vi "DMM Measure Internal Resistance.vi"(0 "instrument handle":refnum<k15>, 5 "V1 (V)":dbl, 11 "error in":errorcluster) -> (4 "instrument handle out":refnum<k15>, 6 "Diode Voltage (V)":dbl, 8 "V2 (V)":dbl, 10 "Internal Resistance (Ohm)":dbl, 15 "error out":errorcluster)   [LabVIEW 2026]
doc: "Measures the cell's internal resistance with the NI-DMM diode function: reads Diode Voltage (1 mA source, mean of 5 readings), then DC volts again (V2, mean of 10 readings at high input impedance), and computes IR = (Diode Voltage - (V1 + V2)/2) / 0.001 Ohm. IR is +Inf when the diode reading is over-range or 4.0 V or more. A driver over-range warning is not passed on as an error. Leaves the DMM configured for DC volts; does not open or close the session."
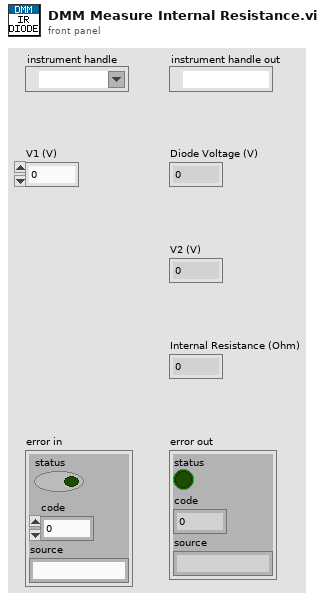
[diagram p1: front panel]
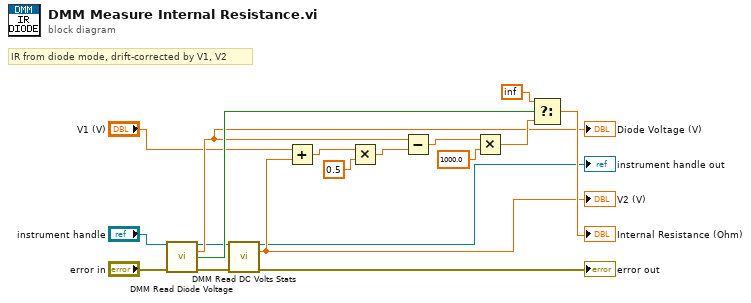
[diagram p0: block diagram]
diagram:
  # "IR from diode mode, drift-corrected by V1, V2"
  n1 = call "DMM Read Diode Voltage.vi"("instrument handle"="instrument handle", "error in"="error in") -> ("instrument handle out"=w4:refnum<k15>, "Diode Voltage (V)"=w5:dbl, "Over Range?"=w6:bool, "error out"=w7:errorcluster)  [unwired: 10 in]
  "Diode Voltage (V)" <- w5
  n2 = call "DMM Read DC Volts Stats.vi"("instrument handle"=w4, "error in"=w7) -> ("instrument handle out"=→"instrument handle out":refnum<k15>, "Mean (V)"=w9:dbl, "error out"=→"error out":errorcluster)  [unwired: 10 in, 1 out]
  "V2 (V)" <- w9
  n3 = Add(x="V1 (V)", y=w9) -> (x+y=w11:dbl)
  n4 = Multiply(x=w11, y=0.5 ("half")) -> (x*y=w13:dbl)
  n5 = Subtract(x=w5, y=w13) -> (x-y=w14:dbl)
  n6 = Multiply(x=w14, y=1000.0 ("1 / 1 mA")) -> (x*y=w16:dbl)
  n7 = Select(t=inf, s=w6, f=w16) -> (s? t:f=→"Internal Resistance (Ohm)":dbl)
